vi "S_ASD Each Signal SAVE_MS VI.vi"(7 "Peak Array":T3, 8 "error in":errorcluster, 9 "S Table C1":T4, 10 "Region raw data":dbl[](array[numeric]), 11 "S_save C":T1) -> (0 "error out":errorcluster, 2 "Raw data 2":dbl[](graph), 3 "S Anal":cluster{string[], string[], string[]})   [LabVIEW 2018]
uses:
  <vilib>/Utility/file.llb/Write Delimited Spreadsheet (DBL).vi
  <vilib>/Analysis/NI_AALBase.lvlib
panel:
  out "S#":i32
  out "Signal#Sum":i32
  out "Histogram Graph":T2(graph) caption="ヒストグラムグラフ"
  out "SS end":i32
  out "SS start":i32
  out "S End":i32[](array[numeric])
  out "S Start":i32[](array[numeric])
  out "サイズ":i32
  out "SR END":i32
  out "SR Start":i32
  out "A New folder":string
  out "data point":i32[](array[numeric])
  out "LL Retention time":dbl
  out "R Peak location":i32[](array[numeric])
  out "Rigon#":i32
  out "PSX Pass":path
  out "S datapoint":i32
  out "部分配列":dbl[](array[numeric])
  out "Filename":path
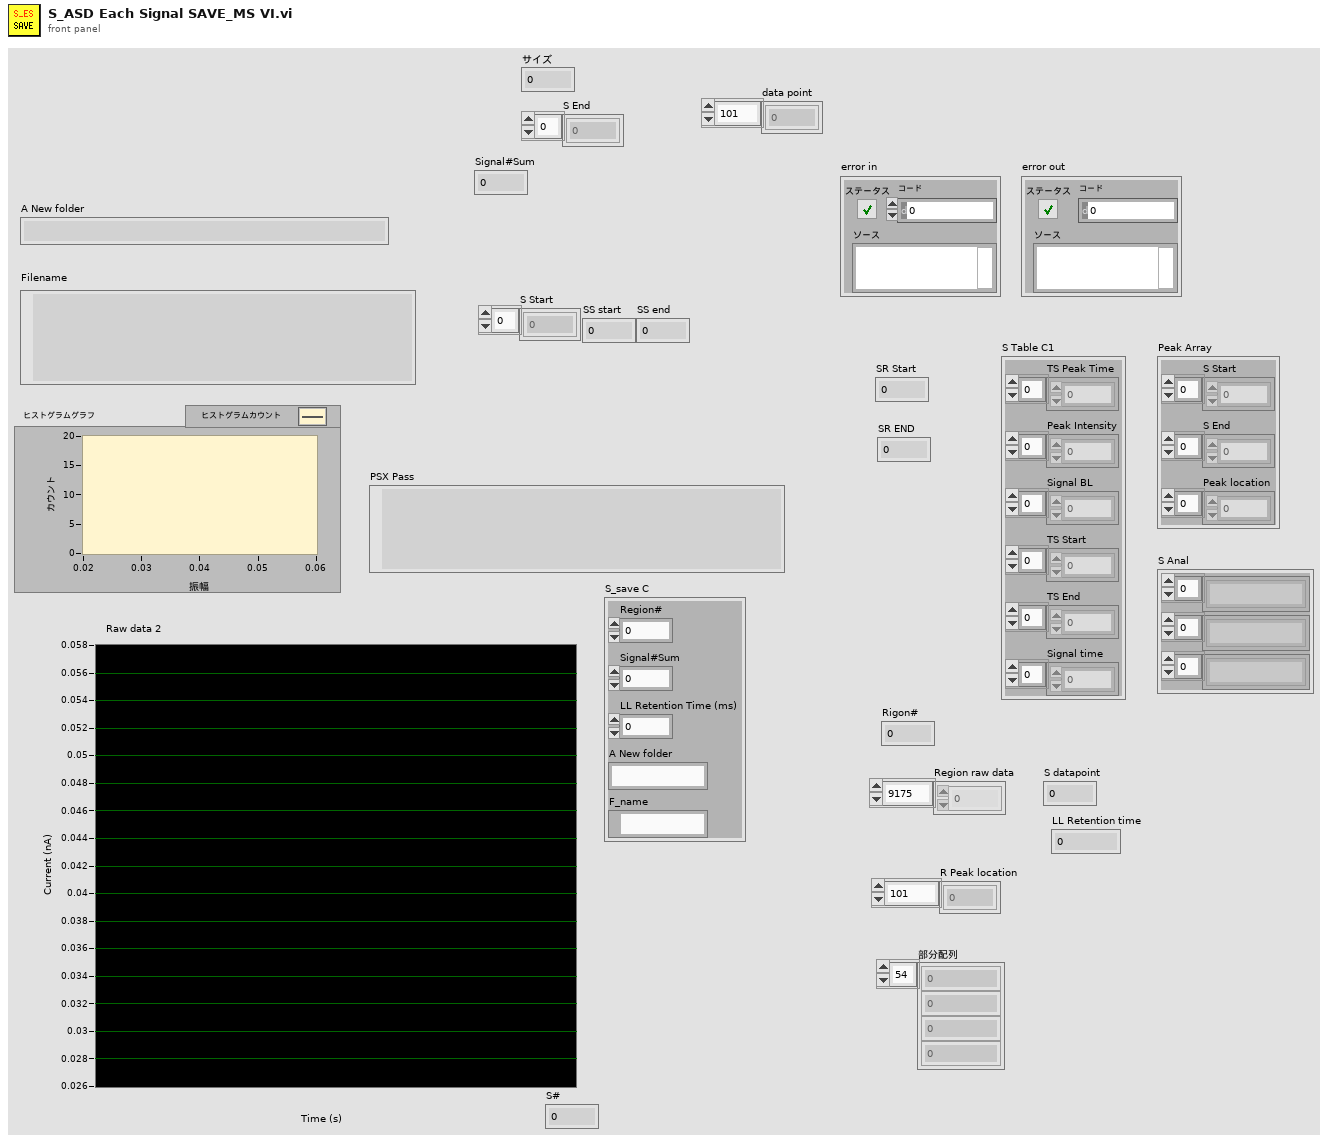
[diagram p1: front panel]
types:
  T1 = cluster{"Region#":i32, "Signal#Sum":i32, "LL Retention Time (ms)":dbl, "A New folder":string, "F_name":path}
  T2 = cluster{"X Values":dbl[], "Histogram: h(x)":i32[]}
  T3 = cluster{"S Start":i32[], "S End":i32[], "Peak location":i32[]}
  T4 = cluster{"TS Peak Time":dbl[], "Peak Intensity":dbl[], "Signal BL":dbl[], "TS Start":dbl[], "TS End":dbl[], "Signal time":dbl[]}
  T5 = cluster{"Size":string, "SH1":string, "SH2":string}
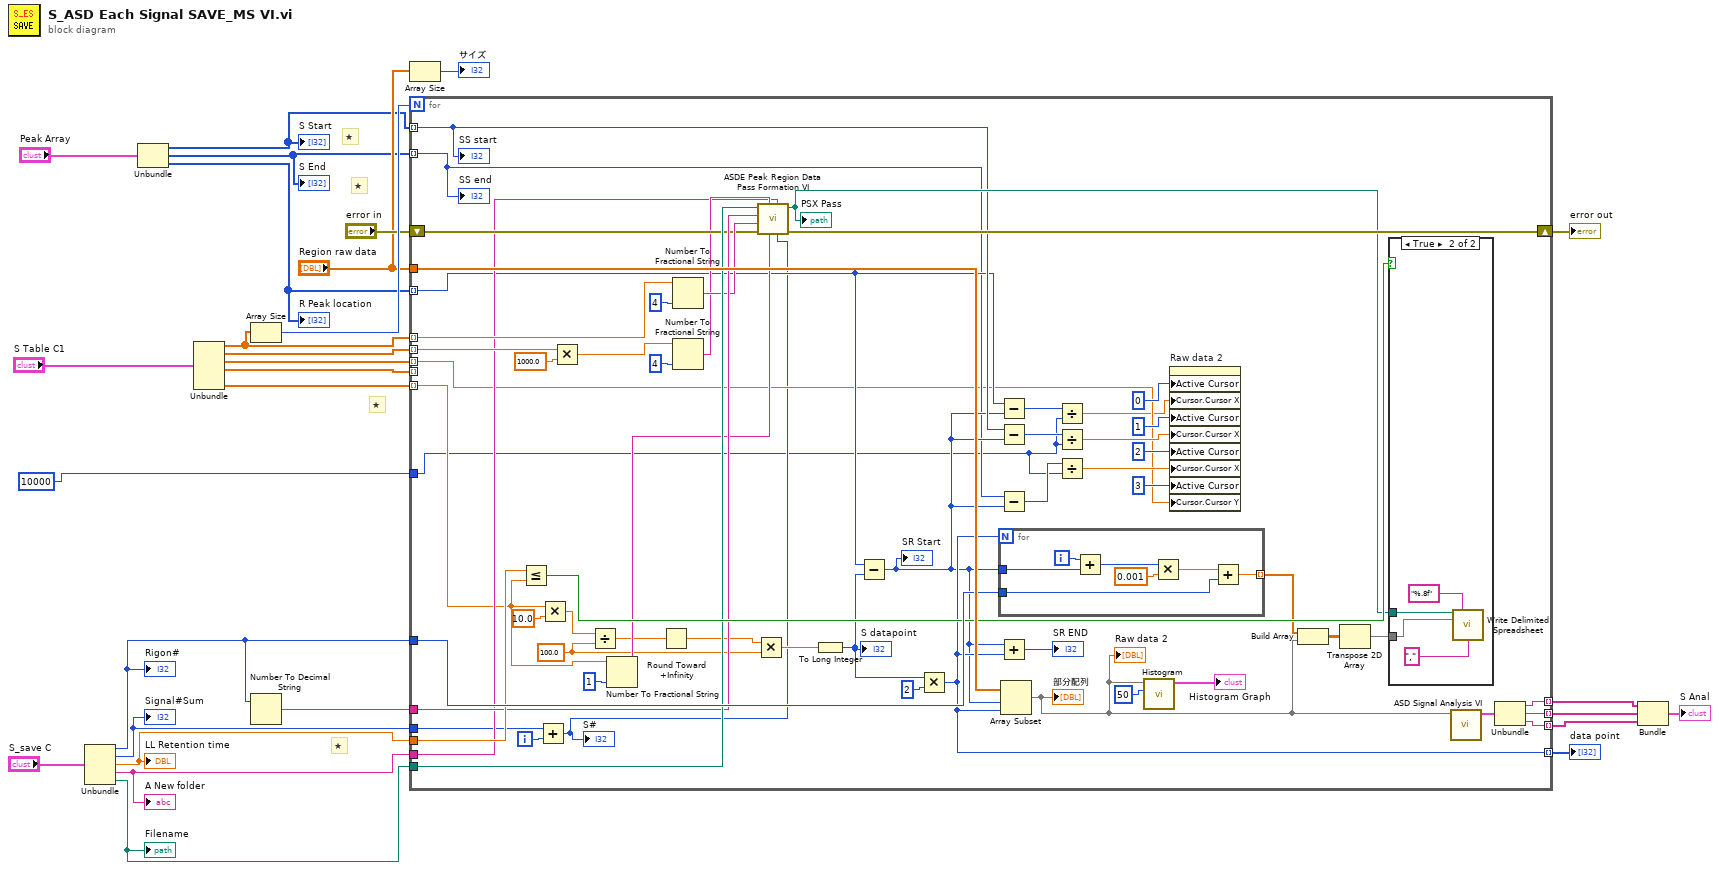
[diagram p0: block diagram]
diagram:
  # "★"
  # "★"
  # "★"
  # "★"
  n1 = Unbundle("S_save C") -> ("Region#"=w5:i32, "Signal#Sum"=w2:i32, "LL Retention Time (ms)"=w4:dbl, "A New folder"=w6:string, "F_name"=w3:path)
  "Filename" <- w3
  "Rigon#" <- w5
  "LL Retention time" <- w4
  "A New folder" <- w6
  "Signal#Sum" <- w2
  n2 = Unbundle("Peak Array") -> ("S Start"=w11:i32[], "S End"=w10:i32[], "Peak location"=w14:i32[])
  "R Peak location" <- w14
  "S Start" <- w11
  "S End" <- w10
  n3 = Unbundle("S Table C1") -> ("TS Peak Time"=w26:dbl[], "Peak Intensity"=w24:dbl[], "Signal BL"=w8:dbl[], "TS Start"=w16:dbl[], "Signal time"=w23:dbl[])  [unwired: 1 out]
  n4 = Array Size(array=w26) -> (size(s)=w27:i32)
  n5 = Number To Decimal String(number=w5) -> (decimal integer string=w25:string)  [unwired: 1 in]
  n6 = Array Size(array="Region raw data") -> (size(s)=→"サイズ":i32)
  n7 = for {
    N: w27 -> [_]
    tunnel: w3 -> [w71]
    tunnel: "Region raw data" -> [w88]
    tunnel: w26 -> [w87] mode=indexing
    tunnel: w25 -> [w70]
    tunnel: w24 -> [w85] mode=indexing
    tunnel: w23 -> [w57] mode=indexing
    tunnel: w14 -> [w45] mode=indexing
    tunnel: w5 -> [w80]
    tunnel: w4 -> [w77]
    shift-right: [w67] -> w21
    shift-left: "error in" -> [w68]
    tunnel: [w74] -> w20 mode=indexing
    tunnel: [w73] -> w19 mode=indexing
    tunnel: [w72] -> w18 mode=indexing
    tunnel: w6 -> [w63]
    tunnel: w16 -> [_] mode=indexing
    tunnel: w11 -> [w49] mode=indexing
    tunnel: w10 -> [w40] mode=indexing
    tunnel: [w52] -> w9 mode=indexing
    tunnel: w8 -> [w37] mode=indexing
    tunnel: w2 -> [w31]
    tunnel: 10000 ("y") -> [w29]
    i -> [w32]
    w58 = 100.0 ("y")
    n8 = Less Or Equal?(x=w77, y=w57) -> (x <= y?=w76:bool)
    n9 = Add(x=w31, y=w32) -> (x+y=w30:i32)
    "S#" <- w30
    n10 = Multiply(x=w57, y=10.0) -> (x*y=w61:dbl)
    n11 = Multiply(x=w85, y=1000.0) -> (x*y=w84:dbl)
    n12 = Divide(x=w61, y=w58) -> (x/y=w60:dbl)
    n13 = Number To Fractional String(number=w57, precision (6)=i16 1 ("精度（6）")) -> (F-format string=w64:string)  [unwired: 2 in]
    n14 = Round Toward +Infinity(x=w60) -> (ceil(x): smallest int >= x=w59:dbl)
    n15 = Number To Fractional String(number=w87, precision (6)=i16 4 ("精度（6）")) -> (F-format string=w69:string)  [unwired: 2 in]
    n16 = Number To Fractional String(number=w84, precision (6)=i16 4 ("精度（6）")) -> (F-format string=w65:string)  [unwired: 2 in]
    n17 = Multiply(x=w59, y=w58) -> (x*y=w56:dbl)
    n18 = call "ASDE Peak Region Data Pass Formation VI.vi"("S#"=w30, "A New folder"=w63, "T (ms)"=w64, "I (pA)"=w65, "error in"=w68, "Signal P"=w69, "N #"=w70, "Filename"=w71) -> ("error out"=w67:errorcluster, "PSX Pass"=w66:path)  [unwired: 2 in]
    "PSX Pass" <- w66
    n19 = To Long Integer(number=w56) -> (32bit integer=w54:i32)
    "S datapoint" <- w54
    n20 = Subtract(x=w45, y=w54) -> (x-y=w41:i32)
    "SR Start" <- w41
    n21 = Multiply(x=w54, y=2) -> (x*y=w52:i32)
    n22 = Subtract(x=w45, y=w41) -> (x-y=w43:i32)
    n23 = Subtract(x=w49, y=w41) -> (x-y=w46:i32)
    n24 = Subtract(x=w40, y=w41) -> (x-y=w42:i32)
    n25 = for {
      N: w52 -> [_]
      tunnel: [w93] -> w51 mode=indexing
      tunnel: w80 -> [w96]
      tunnel: w41 -> [w95]
      i -> [w99]
      n26 = Add(x=w99, y=w95) -> (x+y=w97:i32)
      n27 = Multiply(x=w97, y=0.001) -> (x*y=w94:dbl)
      n28 = Add(x=w94, y=w96) -> (x+y=w93:dbl)
    }
    n29 = Add(x=w41, y=w52) -> (x+y=→"SR END":i32)
    n30 = Array Subset(array=w88, index=w41, length=w52) -> (w33:dbl[])
    "部分配列" <- w33
    "Raw data 2" <- w33
    n31 = Divide(x=w43, y=w29) -> (x/y=w36:dbl)
    n32 = Divide(x=w46, y=w29) -> (x/y=w44:dbl)
    n33 = Divide(x=w42, y=w29) -> (x/y=w39:dbl)
    n34 = call <vilib>:"Histogram.vi"("intervals"=50, "X"=w33) -> ("Histogram Graph"=→"Histogram Graph":T2)  [unwired: 6 in, 3 out]
    n35 = property on="Raw data 2" class="WFGraph (strict)"("Active Cursor"=u32 0 ("アクティブカーソル"), "Cursor.Cursor X"=w36, "Active Cursor"=u32 1 ("アクティブカーソル"), "Cursor.Cursor X"=w44, "Active Cursor"=u32 2 ("アクティブカーソル"), "Cursor.Cursor X"=w39, "Active Cursor"=u32 3 ("アクティブカーソル"), "Cursor.Cursor Y"=w37) -> ()  [unwired: 2 in, 2 out]
    n36 = Build Array(w51, w33) -> (w79:dbl[][])
    n37 = Transpose 2D Array(2D array=w79) -> (transposed array=w78:dbl[][])
    n38 = case shown="True" w76 {
      tunnel: w66 -> [_ w92]
      tunnel: w78 -> [_ w91]
      frame False {
      }
      frame True {
        n39 = call-poly <vilib>:"Write Delimited Spreadsheet.vi"("file path (dialog if empty)"=w92, "format (%.3f)"="%.8f", "2D data"=w91, "delimiter (\\t)"="," ("delimiter (\\t)")) -> ()  [unwired: 10 in, 2 out]
      }
    }
    n40 = call "ASD Signal Analysis VI.vi"("S txt"=w33) -> ("S Analysis"=w75:T5)  [unwired: 8 in, 2 out]
    n41 = Unbundle(w75) -> ("Size"=w74:string, "SH1"=w73:string, "SH2"=w72:string)
    "SS start" <- w49
    "SS end" <- w40
  }
  "error out" <- w21
  "data point" <- w9
  n42 = Bundle(w20, w19, w18) -> (→"S Anal":cluster{string[], string[], string[]})  [unwired: 1 in]
